vi "RP1210 Read Version.vi"(8 "error in (no error)":errorcluster) -> (0 "error out":errorcluster, 1 "fpchAPIMajorVersion":string, 2 "fpchDLLMinorVersion":string, 3 "fpchDLLMajorVersion":string, 5 "fpchAPIMinorVersion":string)   [LabVIEW 2020, in "cansub_rp1210.lvlib"]
doc: "void __stdcall RP1210_ReadVersion(char *fpchDLLMajorVersion, char *fpchDLLMinorVersion,\n char *fpchAPIMajorVersion, char *fpchAPIMinorVersion);"
uses:
  cansub_rp1210.lvlib
  cansub_lv64.dll
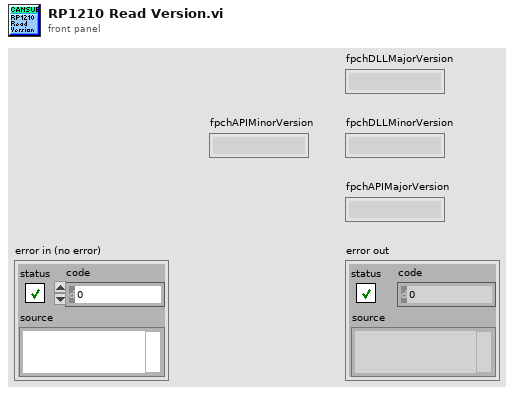
[diagram p1: front panel]
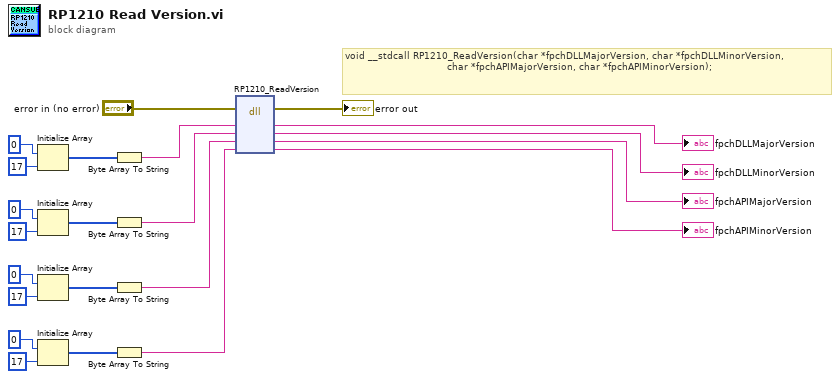
[diagram p0: block diagram]
diagram:
  # "void __stdcall RP1210_ReadVersion(char *fpchDLLMajorVersion, char *fpchDLLMinorVersion,\n                                  char *fpchAPIMajorVersion, char *fpchAPIMinorVersion);"
  n1 = Initialize Array(u8 0 ("element"), 17 ("dimension size")) -> (w22:u8[])
  n2 = Initialize Array(u8 0 ("element"), 17 ("dimension size")) -> (w17:u8[])
  n3 = Initialize Array(u8 0 ("element"), 17 ("dimension size")) -> (w12:u8[])
  n4 = Initialize Array(u8 0 ("element"), 17 ("dimension size")) -> (w7:u8[])
  n5 = Byte Array To String(unsigned byte array=w22) -> (string=w21:string)
  n6 = Byte Array To String(unsigned byte array=w17) -> (string=w16:string)
  n7 = Byte Array To String(unsigned byte array=w12) -> (string=w11:string)
  n8 = Byte Array To String(unsigned byte array=w7) -> (string=w6:string)
  n9 = dll-call lib="C:/cansub-lv/library/cansub_lv*.*" fn="RP1210_ReadVersion"(error in="error in (no error)", "fpchDLLMajorVersion"=w21, "fpchDLLMinorVersion"=w16, "fpchAPIMajorVersion"=w11, "fpchAPIMinorVersion"=w6) -> (error out=→"error out":errorcluster, "fpchDLLMajorVersion"=→"fpchDLLMajorVersion":string, "fpchDLLMinorVersion"=→"fpchDLLMinorVersion":string, "fpchAPIMajorVersion"=→"fpchAPIMajorVersion":string, "fpchAPIMinorVersion"=→"fpchAPIMinorVersion":string)  [unwired: 3 in, 1 out]
